vi "HostMem Create.vi"(8 "error in (no error)":errorcluster, 11 "AllocType":T1) -> (0 "error out":errorcluster, 3 "HostMem":refnum<class "HostMem.lvclass">)   [LabVIEW 2020, in "OpenLvVision_OpenCv.lvlib" / "Cuda.lvlib" / "HostMem.lvclass"]
doc: "Object by Reference!\nCreates an empty host memory"
uses:
  HostMem.lvclass
  C:/Users/lukas/Documents/OpenLvVision_OpenCv/SourceCode/LabView/OpenLvVision_OpenCv/_LvHelpers/EdvrObject/EdvrObject.lvclass
  _LvHelpers/EdvrObject/TypeDef/Edvr.ctl
  _LvHelpers/EdvrObject/EdvrObject.lvclass/EdvrObject.ctl
  _LvHelpers/EdvrObject/EdvrObject.lvclass
  OpenLvVision_OpenCv.lvlib
  Dlls/OlvOpenCvWrapper.dll
  <vilib>/ErrorRing/Error Ring.xnode
  <vilib>/Utility/error.llb/Error Cluster From Error Code.vi
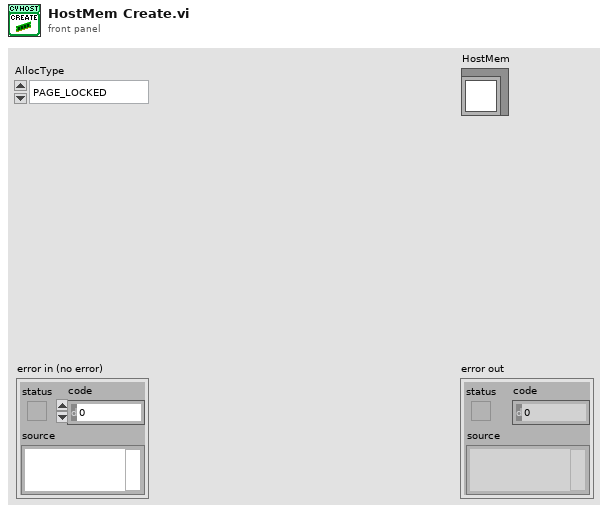
[diagram p1: front panel]
types:
  T1 = typedef "OpenLvVision_OpenCv.lvlib/AllocType" = enum16{"PAGE_LOCKED", "SHARED", "WRITE_COMBINED"}
  T2 = typedef "OpenLvVision_OpenCv.lvlib/EdvrObject.lvclass/Edvr.ctl" = refnum<data-value>
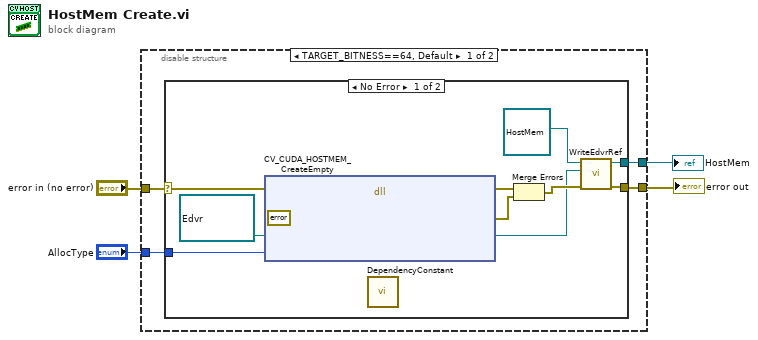
[diagram p0: block diagram]
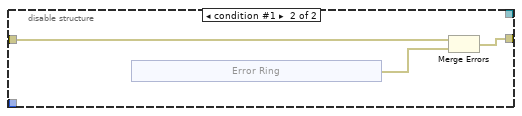
[diagram p3: hidden frame]
diagram:
  n1 = disable-structure shown="TARGET_BITNESS==64, Default" {
    disable-tunnel: "error in (no error)" -> [w8 w22]
    disable-tunnel: [w7 _] -> w3
    disable-tunnel: [w6 w23] -> w2
    disable-tunnel: "AllocType" -> [w5 _]
    frame condition #0 (active) {
      n2 = case shown="No Error" w8 {
        selector: w8 -> [w12 w20]
        tunnel: [w19 w20] -> w6
        tunnel: [w18 _] -> w7
        tunnel: w5 -> [w9 _]
        frame No Error {
          n3 = dll-call lib="C:/Users/lukas/Documents/OpenLvVision_OpenCv/SourceCode/LabView/OpenLvVision_OpenCv/Dlls/OlvOpenCvWrapper.dll" fn="CV_CUDA_HOSTMEM_CreateEmpty"(error in=w12, "Error"=errorcluster {"status"=FALSE, "code"=0, "source"=""} ("error out"), "edvrRef"=T2 refnum ("Edvr"), "allocType"=w9) -> (error out=w16:errorcluster, "Error"=w15:errorcluster, "edvrRef"=w11:T2)  [unwired: 4 in, 1 out]
          n4 = call "DependencyConstant.vi"() -> ()  [unwired: 12 in]
          n5 = Merge Errors(w16, w15) -> (w13:errorcluster)
          n6 = call "WriteEdvrRef.vi"("error in (no error)"=w13, "Edvr"=w11, "EdvrObject in"=refnum<class "HostMem.lvclass"> refnum ("OpenLvVision_OpenCv.lvlib:HostMem")) -> ("error out"=w19:errorcluster, "EdvrObject out"=w18:refnum<class "HostMem.lvclass">)  [unwired: 7 in]
        }
        frame Error {
        }
      }
    }
    frame condition #1 {
      n7 = xnode "Error Ring"() -> ("error out"=w21:errorcluster)
      n8 = Merge Errors(w22, w21) -> (w23:errorcluster)
    }
  }
  "error out" <- w2
  "HostMem" <- w3
